vi "UpdateUI.vi"(8 "error in":errorcluster, 9 "Control Data":variant, 10 "Action":string, 11 "UI_Manager in":refnum<class "UI_Library.lvclass">) -> (0 "error out":errorcluster, 3 "UI_Manager out":refnum<class "UI_Library.lvclass">)   [LabVIEW 2018, in "UI_Library.lvlib" / "UI_Library.lvclass"]
doc: "Handle the UI messages."
uses:
  UI_Library.lvclass
  UI_Library.lvclass/UI_Library.ctl
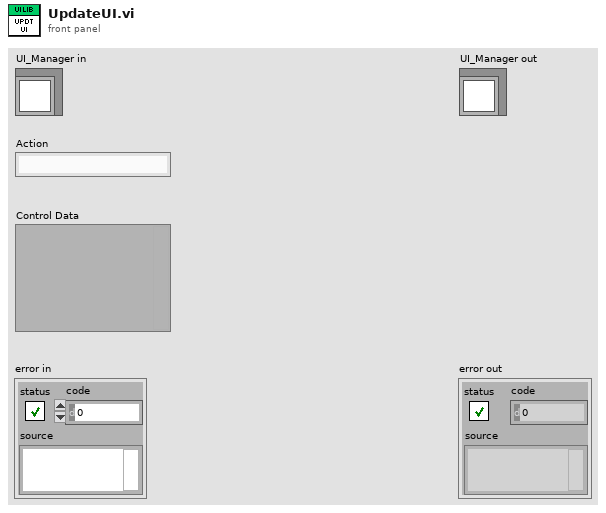
[diagram p1: front panel]
types:
  T1 = cluster{"Ctl_Refnum":refnum<vi>, "Found":bool, "Control Data":variant, "error out":errorcluster}
  T2 = enum8{"Enabled", "Disabled", "Disabled and Grayed Out"}
  T3 = typedef "UI_Library.lvlib/UI_RefCluster.ctl" = cluster{"UI Ctrl Names":string[], "UI Ctrl DataType":T4[], "UI Ctrl Refs":refnum<vi>[]}
  T4 = typedef "NI_Data Type.lvlib/Data Type.ctl" = enum8{"Invalid Type", "Void", "I8", "I16", "I32", "I64", "U8", "U16", "U32", "U64", "Single Float", "Double Float", "Extended Float", "Single Complex", "Double Complex", "Extended Complex", "Enum U8", "Enum U16", "Enum U32", "Enum U64", "Single Float With Unit", "Double Float With Unit", "Extended Float With Unit", "Single Complex with Unit", "Double Complex with Unit", "Extended Complex with Unit", "Boolean", "String", "Path", "Picture", "Tag", "Array", "Cluster", "Variant", "LV Variant", "Waveform", "Timestamp", "Digital Waveform", "Digital Data", "ExpressData", "Refnum", "External Data", "VI", "Poly VI", "LabVIEW Class Instance", "Fixed Point", "Set Collection", "Map Collection"}
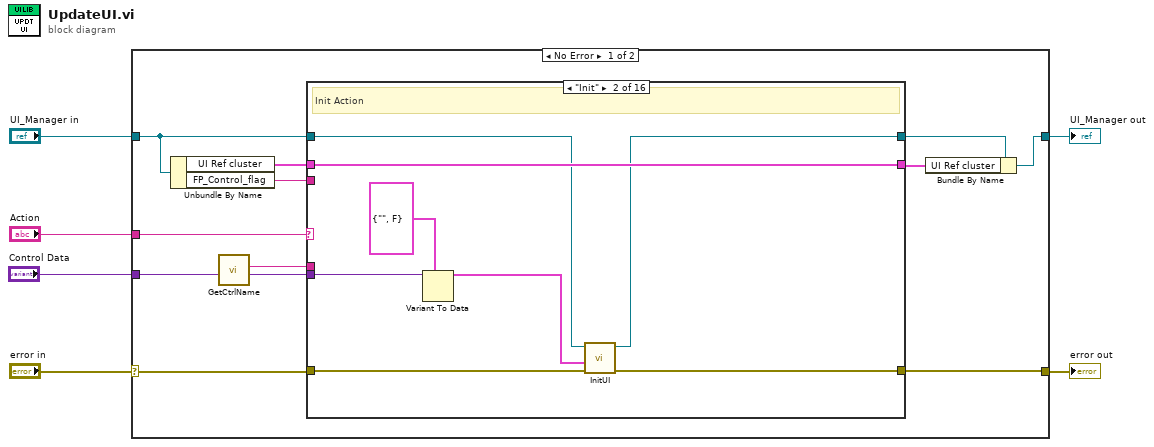
[diagram p0: block diagram]
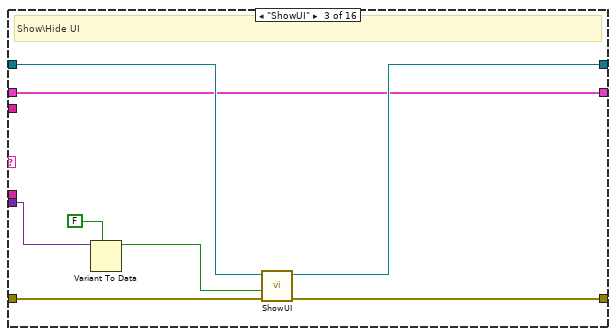
[diagram p3: hidden frame]
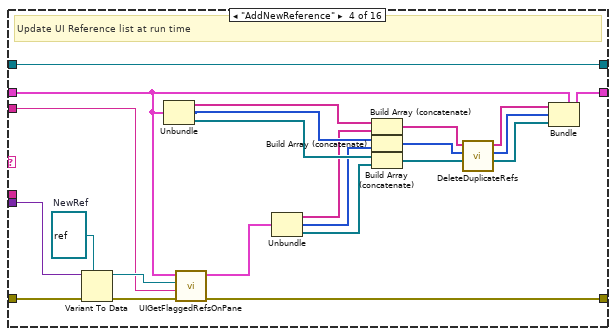
[diagram p4: hidden frame]
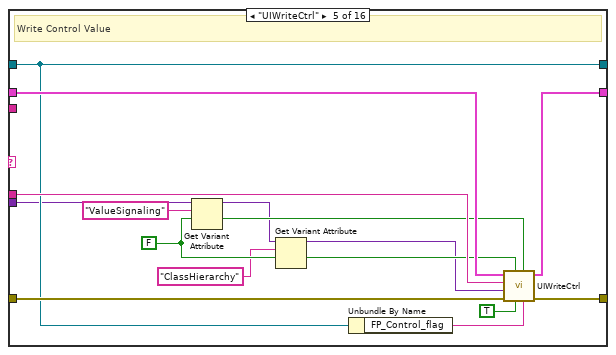
[diagram p5: hidden frame]
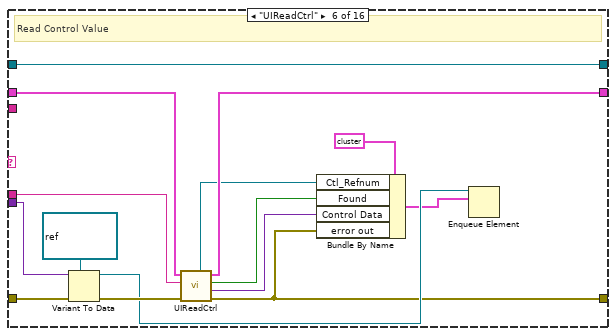
[diagram p6: hidden frame]
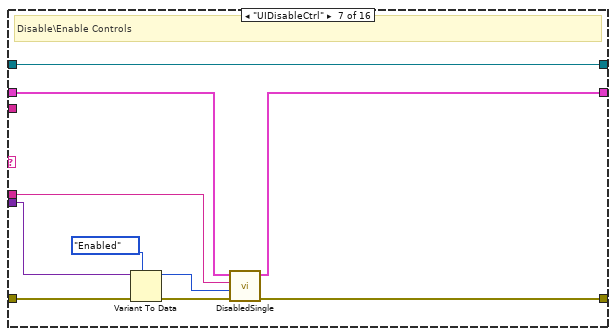
[diagram p7: hidden frame]
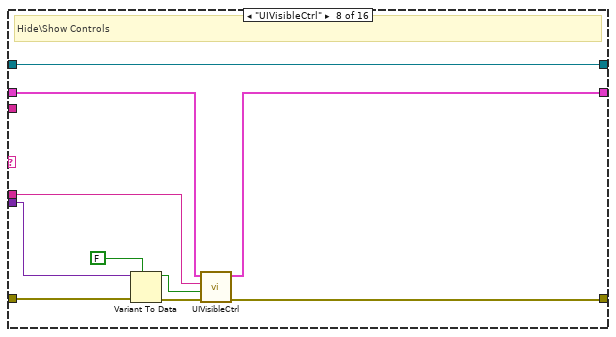
[diagram p8: hidden frame]
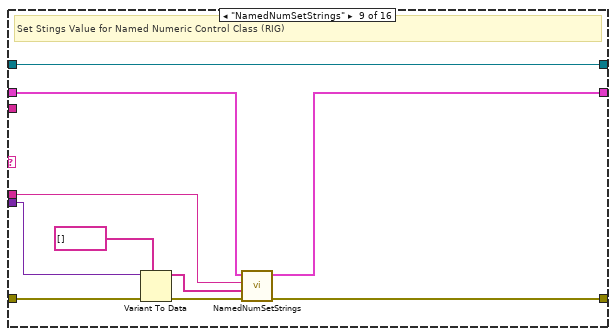
[diagram p9: hidden frame]
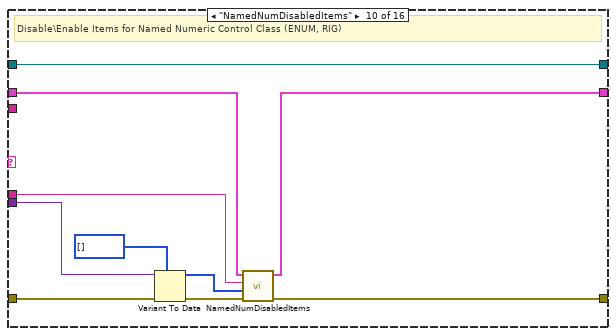
[diagram p10: hidden frame]
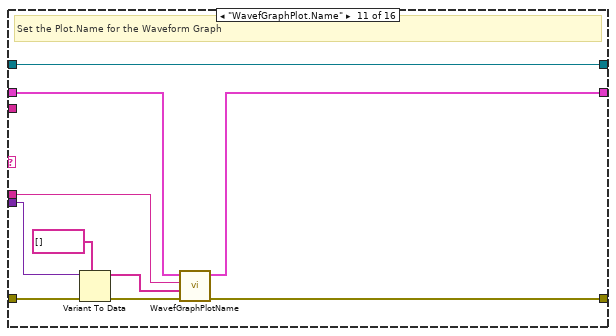
[diagram p11: hidden frame]
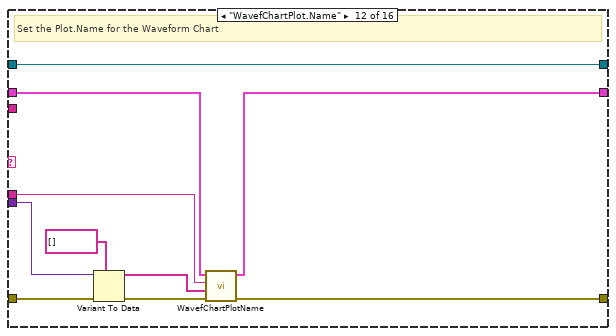
[diagram p12: hidden frame]
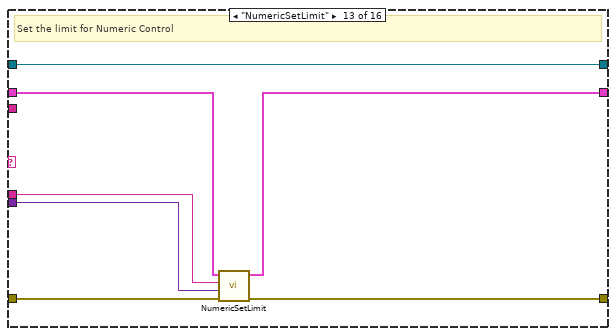
[diagram p13: hidden frame]
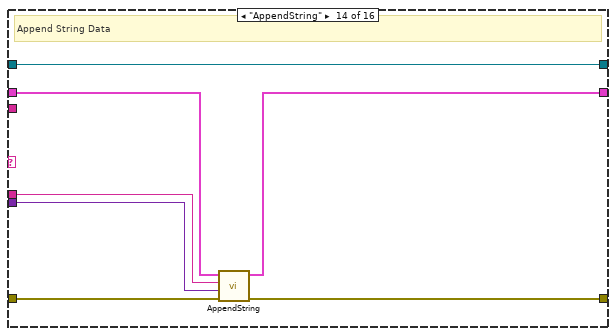
[diagram p14: hidden frame]
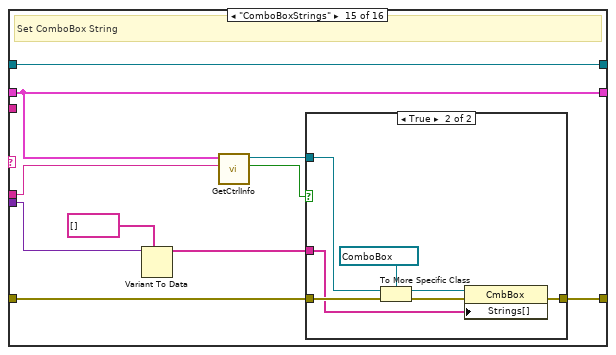
[diagram p15: hidden frame]
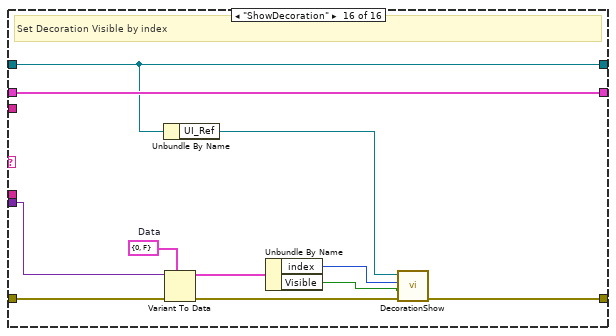
[diagram p17: hidden frame]
diagram:
  n1 = case shown="No Error" "error in" {
    selector: "error in" -> [w12 w196]
    tunnel: [w11 w196] -> w5
    tunnel: [w13 w195] -> w3
    tunnel: "UI_Manager in" -> [w8 w195]
    tunnel: "Control Data" -> [w10 _]
    tunnel: "Action" -> [w9 _]
    frame No Error {
      n2 = Unbundle By Name(w8) -> ("UI Ref cluster"=w16:T3, "FP_Control_flag"=w7:string)
      n3 = call "GetCtrlName.vi"("Control Data"=w10) -> ("Ctrl Label"=w18:string, "Data"=w17:variant)  [unwired: 5 in, 1 out]
      n4 = case shown="\"Init\"" w9 {
        tunnel: w8 -> [w21 w23 w34 w60 w71 w91 w97 w108 w117 w127 w139 w148 w156 w162 w175 w184]
        tunnel: [w19 w29 w33 w56 w73 w88 w96 w107 w113 w126 w138 w147 w155 w163 w167 w193] -> w14
        tunnel: w18 -> [_ _ _ _ w75 w90 w94 w106 w116 w125 w136 w144 w154 w161 w170 _]
        tunnel: w17 -> [_ w28 w32 w58 w68 w86 w99 w109 w119 w129 w135 w150 w157 w160 w169 w194]
        tunnel: w12 -> [w20 w26 w37 w59 w76 w89 w100 w110 w120 w130 w141 w151 w158 w165 w168 w192]
        tunnel: [w20 w25 w36 w38 w72 w77 w95 w103 w114 w123 w137 w146 w153 w164 w166 w190] -> w11
        tunnel: w16 -> [w19 w29 w33 w42 w74 w83 w92 w102 w112 w122 w133 w143 w152 w159 w167 w193]
        tunnel: [w21 w24 w35 w60 w71 w91 w97 w108 w117 w127 w139 w148 w156 w162 w175 w184] -> w15
        tunnel: w7 -> [_ _ _ w41 _ _ _ _ _ _ _ _ _ _ _ _]
        frame Default {
          # "Unknow Action"
        }
        frame "Init" {
          # "Init Action"
          n5 = Variant To Data(type=cluster{"UITitle":string, "HideUI":bool} {"UITitle"="", "HideUI"=FALSE}, Variant=w28) -> (data=w22:cluster{"UITitle":string, "HideUI":bool})  [unwired: 1 in, 1 out]
          n6 = call-dynamic "InitUI.vi"("error in"=w26, "Data"=w22, "UI_Library in"=w23) -> ("error out"=w25:errorcluster, "UI_Library out"=w24:refnum<class "UI_Library.lvclass">)  [unwired: 7 in]
        }
        frame "ShowUI" {
          # "Show\\Hide UI"
          n7 = Variant To Data(type=FALSE, Variant=w32) -> (data=w30:bool)  [unwired: 1 in, 1 out]
          n8 = call-dynamic "ShowUI.vi"("error in"=w37, "ShowUI"=w30, "UI_Library in"=w34) -> ("error out"=w36:errorcluster, "UI_Library out"=w35:refnum<class "UI_Library.lvclass">)  [unwired: 7 in]
        }
        frame "AddNewReference" {
          w44 = refnum<vi> refnum  # NewRef
          # "Update UI Reference list at run time"
          n9 = Variant To Data(error in=w59, type=w44, Variant=w58) -> (data=w43:refnum<vi>, error out=w40:errorcluster)
          n10 = Unbundle(w42) -> ("UI Ctrl Names"=w57:string[], "UI Ctrl DataType"=w55:T4[], "UI Ctrl Refs"=w54:refnum<vi>[])
          n11 = call "UIGetFlaggedRefsOnPane.vi"("error in"=w40, "Flag"=w41, "VI Ref"=w43, "UI Ref cluster in"=w42) -> ("error out"=w38:errorcluster, "UI Ref cluster out"=w39:T3)  [unwired: 6 in]
          n12 = Unbundle(w39) -> ("UI Ctrl Names"=w51:string[], "UI Ctrl DataType"=w53:T4[], "UI Ctrl Refs"=w52:refnum<vi>[])
          n13 = Build Array (concatenate)(w57, w51) -> (w50:string[])
          n14 = Build Array (concatenate)(w55, w53) -> (w49:T4[])
          n15 = Build Array (concatenate)(w54, w52) -> (w48:refnum<vi>[])
          n16 = call "DeleteDuplicateRefs.vi"("CtrlRefs"=w48, "DataType"=w49, "CtrlNames"=w50) -> ("CtrlRefs out"=w45:refnum<vi>[], "DataType out"=w46:T4[], "CtrlNames out"=w47:string[])  [unwired: 6 in]
          n17 = Bundle(cluster=w42, "UI Ctrl Names"=w47, "UI Ctrl DataType"=w46, "UI Ctrl Refs"=w45) -> (w56:T3)
        }
        frame "UIWriteCtrl" {
          w64 = FALSE
          # "Write Control Value"
          n18 = Get Variant Attribute(Variant=w68, name="ValueSignaling", default value (empty Variant)=w64) -> (duplicate Variant=w62:variant, value=w66:bool)  [unwired: 1 in, 2 out]
          n19 = Get Variant Attribute(Variant=w62, name="ClassHierarchy", default value (empty Variant)=w64) -> (duplicate Variant=w61:variant, value=w65:bool)  [unwired: 1 in, 2 out]
          n20 = Unbundle By Name(w71) -> ("FP_Control_flag"=w70:string)
          n21 = call "UIWriteCtrl.vi"("UI Flag"=w70, "Value Signaling (F)"=w66, "Search Whole Word (T)"=TRUE, "Class_Hierarchy (F)"=w65, "error in"=w76, "Control Value"=w61, "Control Label"=w75, "UI Ref cluster in"=w74) -> ("error out"=w72:errorcluster, "UI Ref cluster out"=w73:T3)  [unwired: 2 in]
        }
        frame "UIReadCtrl" {
          # "Read Control Value"
          n22 = Variant To Data(error in=w89, type=refnum<queue> refnum ("queue out"), Variant=w86) -> (data=w84:refnum<queue>, error out=w87:errorcluster)
          n23 = call "UIReadCtrl.vi"("error in"=w87, "Control Label"=w90, "UI Ref cluster in"=w83) -> ("error out"=w77:errorcluster, "Control Value"=w79:variant, "Found"=w80:bool, "UI Ref cluster out"=w88:T3, "CtrlRef"=w78:refnum<vi>)  [unwired: 4 in]
          n24 = Bundle By Name(cluster=T1 {"Ctl_Refnum"=refnum, "Found"=FALSE, "Control Data"=variant, "error out"={"status"=FALSE, "code"=0, "source"=""}}, "Ctl_Refnum"=w78, "Found"=w80, "Control Data"=w79, "error out"=w77) -> (w81:T1)
          n25 = Enqueue Element(queue=w84, element=w81) -> ()  [unwired: 2 in, 3 out]
        }
        frame "UIDisableCtrl" {
          # "Disable\\Enable Controls"
          n26 = Variant To Data(error in=w100, type=T2."Enabled" ("Disabled"), Variant=w99) -> (data=w93:T2, error out=w98:errorcluster)
          n27 = call "DisabledSingle.vi"("error in"=w98, "Disabled"=w93, "Control Label"=w94, "UI Ref cluster in"=w92) -> ("error out"=w95:errorcluster, "UI Ref cluster out"=w96:T3)  [unwired: 6 in]
        }
        frame "UIVisibleCtrl" {
          # "Hide\\Show Controls"
          n28 = Variant To Data(error in=w110, type=FALSE, Variant=w109) -> (data=w104:bool, error out=w105:errorcluster)
          n29 = call "UIVisibleCtrl.vi"("error in"=w105, "Visible"=w104, "Control Label"=w106, "UI Ref cluster in"=w102) -> ("error out"=w103:errorcluster, "UI Ref cluster out"=w107:T3)  [unwired: 6 in]
        }
        frame "NamedNumSetStrings" {
          # "Set Stings Value for Named Numeric Control Class (RIG)"
          n30 = Variant To Data(error in=w120, type=string[] [], Variant=w119) -> (data=w115:string[], error out=w118:errorcluster)
          n31 = call "NamedNumSetStrings.vi"("error in"=w118, "Strings"=w115, "Control Label"=w116, "UI Ref cluster in"=w112) -> ("error out"=w114:errorcluster, "UI Ref cluster out"=w113:T3)  [unwired: 6 in]
        }
        frame "NamedNumDisabledItems" {
          # "Disable\\Enable Items for Named Numeric Control Class (ENUM, RIG)"
          n32 = Variant To Data(error in=w130, type=i32[] [], Variant=w129) -> (data=w124:i32[], error out=w128:errorcluster)
          n33 = call "NamedNumDisabledItems.vi"("error in"=w128, "Disabled Items"=w124, "Control Label"=w125, "UI Ref cluster in"=w122) -> ("error out"=w123:errorcluster, "UI Ref cluster out"=w126:T3)  [unwired: 6 in]
        }
        frame "WavefGraphPlot.Name" {
          # "Set the Plot.Name for the Waveform Graph"
          n34 = Variant To Data(error in=w141, type=string[] [], Variant=w135) -> (data=w134:string[], error out=w140:errorcluster)
          n35 = call "WavefGraphPlotName.vi"("error in"=w140, "Plot Name"=w134, "Control Label"=w136, "UI Ref cluster in"=w133) -> ("error out"=w137:errorcluster, "UI Ref cluster out"=w138:T3)  [unwired: 6 in]
        }
        frame "WavefChartPlot.Name" {
          # "Set the Plot.Name for the Waveform Chart"
          n36 = Variant To Data(error in=w151, type=string[] [], Variant=w150) -> (data=w145:string[], error out=w149:errorcluster)
          n37 = call "WavefChartPlotName.vi"("error in"=w149, "Plot Name"=w145, "Control Label"=w144, "UI Ref cluster in"=w143) -> ("error out"=w146:errorcluster, "UI Ref cluster out"=w147:T3)  [unwired: 6 in]
        }
        frame "NumericSetLimit" {
          # "Set the limit for Numeric Control"
          n38 = call "NumericSetLimit.vi"("error in"=w158, "Control Value"=w157, "Control Label"=w154, "UI Ref cluster in"=w152) -> ("error out"=w153:errorcluster, "UI Ref cluster out"=w155:T3)  [unwired: 6 in]
        }
        frame "AppendString" {
          # "Append String Data"
          n39 = call "AppendString.vi"("error in"=w165, "Control Value"=w160, "Control Label"=w161, "UI Ref cluster in"=w159) -> ("error out"=w164:errorcluster, "UI Ref cluster out"=w163:T3)  [unwired: 6 in]
        }
        frame "ComboBoxStrings" {
          # "Set ComboBox String"
          n40 = Variant To Data(type=string[] [], Variant=w169) -> (data=w172:string[])  [unwired: 1 in, 1 out]
          n41 = call "GetCtrlInfo.vi"("Ctrl Label"=w170, "UI Ref cluster"=w167) -> ("Found"=w174:bool, "Control out"=w173:refnum<vi>)  [unwired: 8 in]
          n42 = case shown="True" w174 {
            tunnel: w173 -> [_ w177]
            tunnel: w168 -> [w176 w182]
            tunnel: [w176 w183] -> w166
            tunnel: w172 -> [_ w178]
            frame False {
            }
            frame True {
              n43 = To More Specific Class(target class=refnum<vi> refnum ("reference"), reference=w177, error in=w182) -> (specific class reference=w179:refnum<vi>, error out=w181:errorcluster)
              n44 = property on="Property Node" class="CmbBox"(reference=w179, error in=w181, "Strings[]"=w178) -> (error out=w183:errorcluster)  [unwired: 1 out]
            }
          }
        }
        frame "ShowDecoration" {
          w188 = cluster{"index":i32, "Visible":bool} {"index"=0, "Visible"=FALSE}  # Data
          # "Set Decoration Visible by index"
          n45 = Unbundle By Name(w184) -> ("UI_Ref"=w189:refnum<vi>)
          n46 = Variant To Data(error in=w192, type=w188, Variant=w194) -> (data=w187:cluster{"index":i32, "Visible":bool}, error out=w191:errorcluster)
          n47 = Unbundle By Name(w187) -> ("index"=w186:i32, "Visible"=w185:bool)
          n48 = call "DecorationShow.vi"("error in (no error)"=w191, "Visible"=w185, "index"=w186, "VI_Ref"=w189) -> ("error out"=w190:errorcluster)  [unwired: 7 in]
        }
      }
      n49 = Bundle By Name(cluster=w15, "UI Ref cluster"=w14) -> (w13:refnum<class "UI_Library.lvclass">)
    }
    frame Error {
    }
  }
  "error out" <- w5
  "UI_Manager out" <- w3
